vi "WaitTime.vi"(9 "wait time(ms)":u32=100, 11 "error in (no error)":errorcluster caption="error in(no error)") -> (1 "毫秒计时值":u32, 3 "error out":errorcluster)   [LabVIEW 2025]
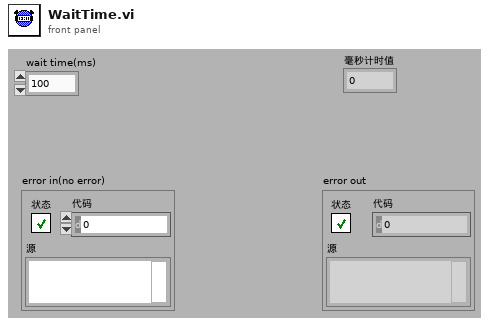
[diagram p1: front panel]
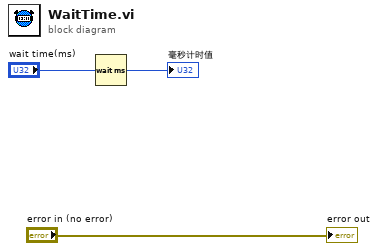
[diagram p0: block diagram]
diagram:
  n1 = Wait (ms)(milliseconds to wait="wait time(ms)") -> (millisecond timer value=→"毫秒计时值":u32)
  "error out" <- "error in (no error)"
